vi "Configure Module.vi"(8 "error in (no error)":errorcluster, 10 "IOV ref in":variant, 11 "Module Template in":refnum<class "9211.lvclass">) -> (0 "error out":errorcluster, 2 "IOV ref out":variant, 3 "Module Template out":refnum<class "9211.lvclass">)   [LabVIEW 2020, in "Modules.lvlib" / "9211.lvclass"]
uses:
  9211.lvclass
  <resource>/objmgr/cRIO.rc
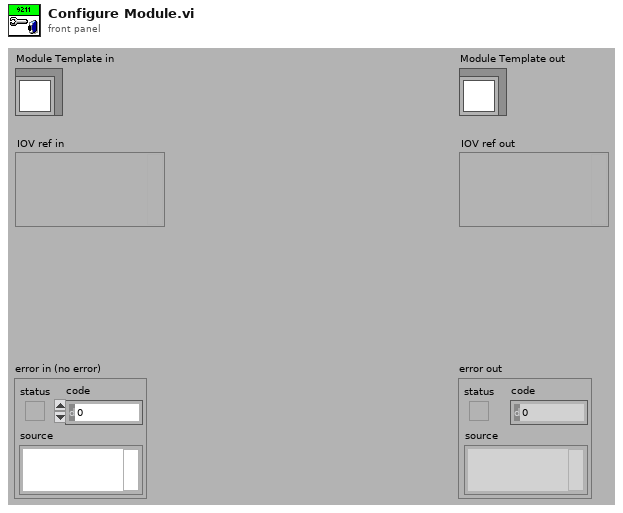
[diagram p1: front panel]
types:
  T1 = cluster{"Degree range":u32, "Thermocouple type":u32}[]
  T2 = cluster{"Degree range":u32, "Thermocouple type":u32}
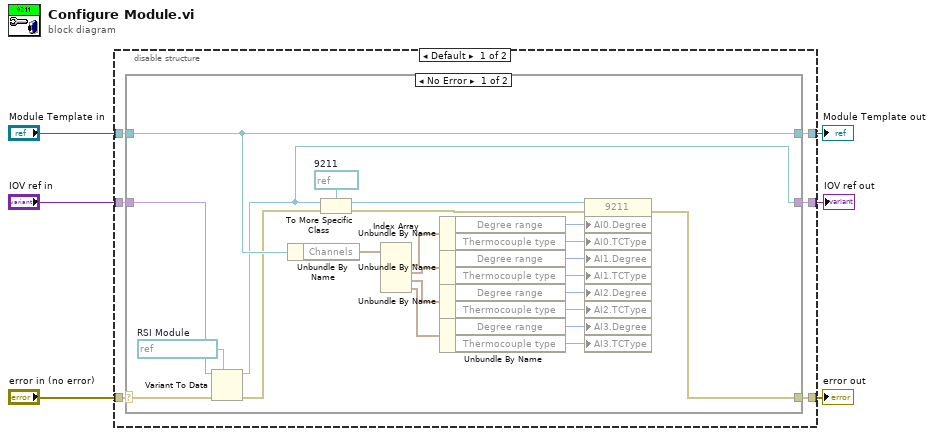
[diagram p0: block diagram]
diagram:
  n1 = disable-structure shown="Default" {
    disable-tunnel: "error in (no error)" -> [w12 w39]
    disable-tunnel: [w11 w39] -> w5
    disable-tunnel: "Module Template in" -> [w10 w41]
    disable-tunnel: [w9 w41] -> w3
    disable-tunnel: "IOV ref in" -> [w8 w40]
    disable-tunnel: [w7 w40] -> w1
    frame condition #0 {
      n2 = case shown="No Error" w12 {
        selector: w12 -> [w34 w38]
        tunnel: [w30 w38] -> w11
        tunnel: [w35 w37] -> w9
        tunnel: w10 -> [w35 w37]
        tunnel: w8 -> [w15 w36]
        tunnel: [w14 w36] -> w7
        frame No Error {
          w13 = refnum<k21> refnum  # RSI Module
          w33 = refnum<k21> refnum  # 9211
          n3 = Variant To Data(error in=w34, type=w13, Variant=w15) -> (data=w14:refnum<k21>, error out=w16:errorcluster)
          n4 = Unbundle By Name(w35) -> ("Channels"=w29:T1)
          n5 = To More Specific Class(target class=w33, reference=w14, error in=w16) -> (specific class reference=w32:refnum<k21>, error out=w31:errorcluster)
          n6 = Index Array(array=w29) -> (element #1=w28:T2, element #2=w19:T2, element #3=w18:T2, element #4=w17:T2)  [unwired: 4 in]
          n7 = Unbundle By Name(w28) -> ("Degree range"=w27:u32, "Thermocouple type"=w26:u32)
          n8 = Unbundle By Name(w19) -> ("Degree range"=w25:u32, "Thermocouple type"=w24:u32)
          n9 = Unbundle By Name(w18) -> ("Degree range"=w23:u32, "Thermocouple type"=w22:u32)
          n10 = Unbundle By Name(w17) -> ("Degree range"=w21:u32, "Thermocouple type"=w20:u32)
          n11 = property class="9211"(reference=w32, error in=w31, "AI0.Degree"=w27, "AI0.TCType"=w26, "AI1.Degree"=w25, "AI1.TCType"=w24, "AI2.Degree"=w23, "AI2.TCType"=w22, "AI3.Degree"=w21, "AI3.TCType"=w20) -> (error out=w30:errorcluster)  [unwired: 1 out]
        }
        frame Error {
        }
      }
    }
    frame condition #1 (active) {
    }
  }
  "error out" <- w5
  "Module Template out" <- w3
  "IOV ref out" <- w1
